vi "Delete_database.vi"(6 "name":string, 8 "error in (no error)":errorcluster caption="错误输入（无错误）", 9 "Item-name":string, 10 "table":string, 11 "Database_access 输入":refnum<class "Database_access.lvclass">) -> (0 "error out":errorcluster caption="错误输出", 3 "Database_access 输出":refnum<class "Database_access.lvclass">)   [LabVIEW 2025, in "Database_access.lvclass"]
uses:
  Database_access.lvclass
  Database_access.lvclass/Database_access.ctl
  <vilib>/addons/database/NI_Database_API.lvlib
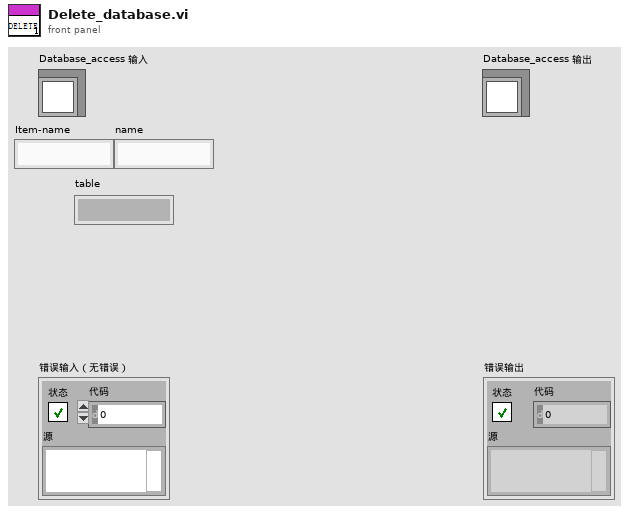
[diagram p1: front panel]
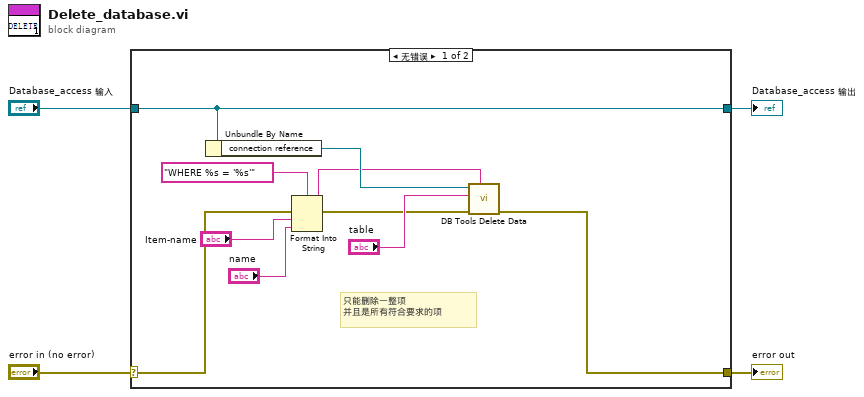
[diagram p0: block diagram]
diagram:
  n1 = case shown="无错误" "error in (no error)" {
    selector: "error in (no error)" -> [w9 w16]
    tunnel: [w11 w16] -> w3
    tunnel: [w14 w15] -> w1
    tunnel: "Database_access 输入" -> [w14 w15]
    frame No Error {
      # "只能删除一整项\n并且是所有符合要求的项"
      n2 = Unbundle By Name(w14) -> ("connection reference"=w13:refnum<k1>)
      n3 = Format Into String(format string="WHERE %s = '%s'" ("格式字符串"), error in=w9, "Item-name", "name") -> (resulting string=w10:string, error out=w8:errorcluster)  [unwired: 1 in]
      n4 = call <vilib>:"DB Tools Delete Data.vi"("condition"=w10, "error in (no error)"=w8, "table"="table", "connection reference"=w13) -> ("error out"=w11:errorcluster)  [unwired: 6 in, 1 out]
    }
    frame Error {
    }
  }
  "error out" <- w3
  "Database_access 输出" <- w1
